vi "ZMQ.Handle Error.vi"(8 "error in (no error)":errorcluster, 11 "RemoteControl.ZMQ in":refnum<class "RemoteControl.ZMQ.lvclass">) -> (0 "error out":errorcluster, 3 "RemoteControl.ZMQ out":refnum<class "RemoteControl.ZMQ.lvclass">)   [LabVIEW 2019, in "RemoteControl.ZMQ.lvlib" / "RemoteControl.ZMQ.lvclass"]
uses:
  RemoteControl.ZMQ.lvclass
  <vilib>/addons/zeromq/zeromq.lvlib
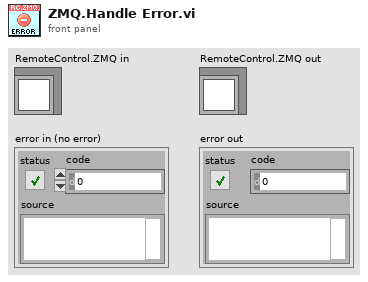
[diagram p1: front panel]
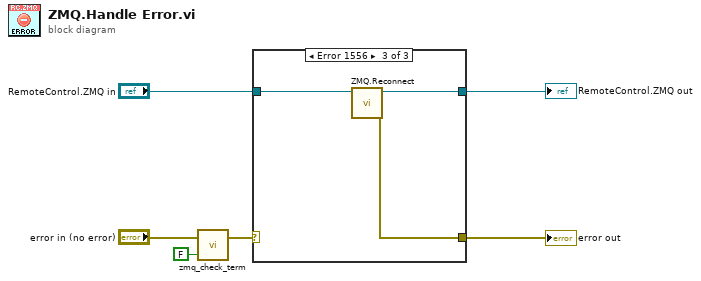
[diagram p0: block diagram]
diagram:
  n1 = call <vilib>:"zmq_check_term.vi"("drop term? (T)"=FALSE, "error in"="error in (no error)") -> ("error out"=w2:errorcluster)  [unwired: 1 out]
  n2 = case shown="Error 1556" w2 {
    selector: w2 -> [w8 w9 _]
    tunnel: [w8 w9 w11] -> w6
    tunnel: [w7 w10 w13] -> w5
    tunnel: "RemoteControl.ZMQ in" -> [w7 w10 w12]
    frame No Error {
    }
    frame Default {
    }
    frame Error {
      n3 = call "ZMQ.Reconnect.vi"("RemoteControl.ZMQ in"=w12) -> ("error out"=w11:errorcluster, "RemoteControl.ZMQ out"=w13:refnum<class "RemoteControl.ZMQ.lvclass">)  [unwired: 9 in]
    }
  }
  "error out" <- w6
  "RemoteControl.ZMQ out" <- w5
